vi "Mark As Changed.vi"(10 "Changed elements":string[](array[string]), 11 "ConfigManager.Text in":refnum<class "ConfigManager.Text.lvclass">) -> (3 "ConfigManager.Text out":refnum<class "ConfigManager.Text.lvclass">)   [LabVIEW 2013, in "CfgManager.Text.lvlib" / "ConfigManager.Text.lvclass"]
uses:
  ConfigManager.Text.lvclass
  ConfigManager.Text.lvclass/ConfigManager.Text.ctl
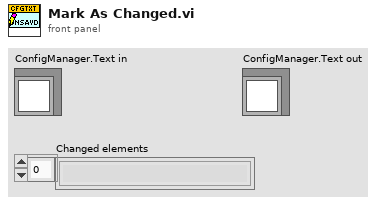
[diagram p1: front panel]
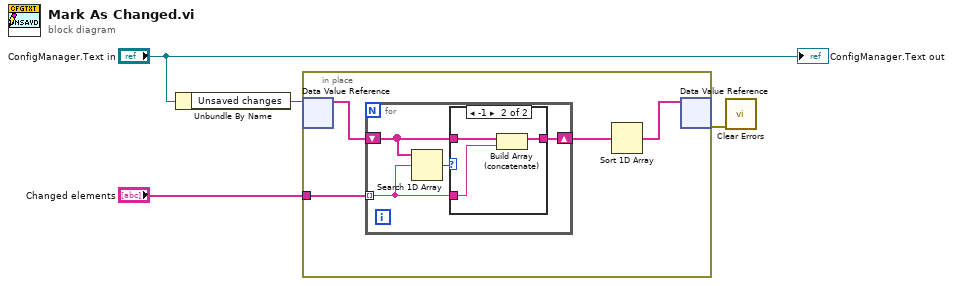
[diagram p0: block diagram]
diagram:
  n1 = Unbundle By Name("ConfigManager.Text in") -> ("Unsaved changes"=w3:refnum<data-value>)
  n2 = in-place {
    in-place-border: "Changed elements" -> [w8]
    n3 = in-place-dvr #1(w3) -> (w6:string[])  [unwired: 1 out]
    n4 = for {
      tunnel: w8 -> [w11] mode=indexing
      shift-right: [w10] -> w7
      shift-left: w6 -> [w12]
      n5 = Search 1D Array(1D array=w12, element=w11) -> (index of element=w9:i32)  [unwired: 1 in]
      n6 = case shown="-1" w9 {
        tunnel: w12 -> [w13 w16]
        tunnel: w11 -> [_ w15]
        tunnel: [w13 w14] -> w10
        frame Default {
        }
        frame -1 {
          n7 = Build Array (concatenate)(w16, w15) -> (w14:string[])
        }
      }
    }
    n8 = Sort 1D Array(array=w7) -> (sorted array=w5:string[])
    n9 = in-place-dvr #1(w5) -> (w1:errorcluster)  [unwired: 1 out]
  }
  n10 = call <vilib>:"Clear Errors.vi"("error in (no error)"=w1) -> ()  [unwired: 6 in, 1 out]
  "ConfigManager.Text out" <- "ConfigManager.Text in"
